vi "ReadAndParseXML.vi"() -> (0 "Mode XML Elements":string, 2 "XML Elements":string[](array[string]))   [LabVIEW 2023, in "GettingStartedWindow.lvlib"]
uses:
  <resource>/modes/FRC/GettingStartedWindow.lvlib
  <resource>/modes/FRC/LocalizedStrings.vi
panel:
  out "error out":errorcluster
  in  "error in (no error)":errorcluster
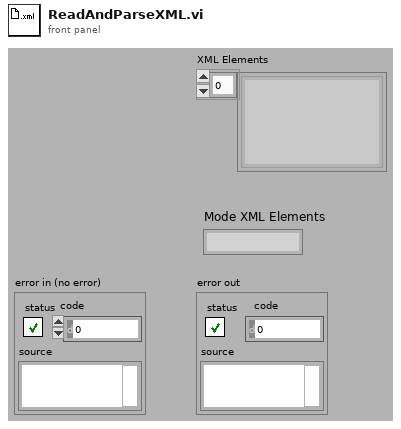
[diagram p1: front panel]
types:
  T1 = enum16{"open", "replace", "create", "open or create", "replace or create", "replace or create with confirmation"}
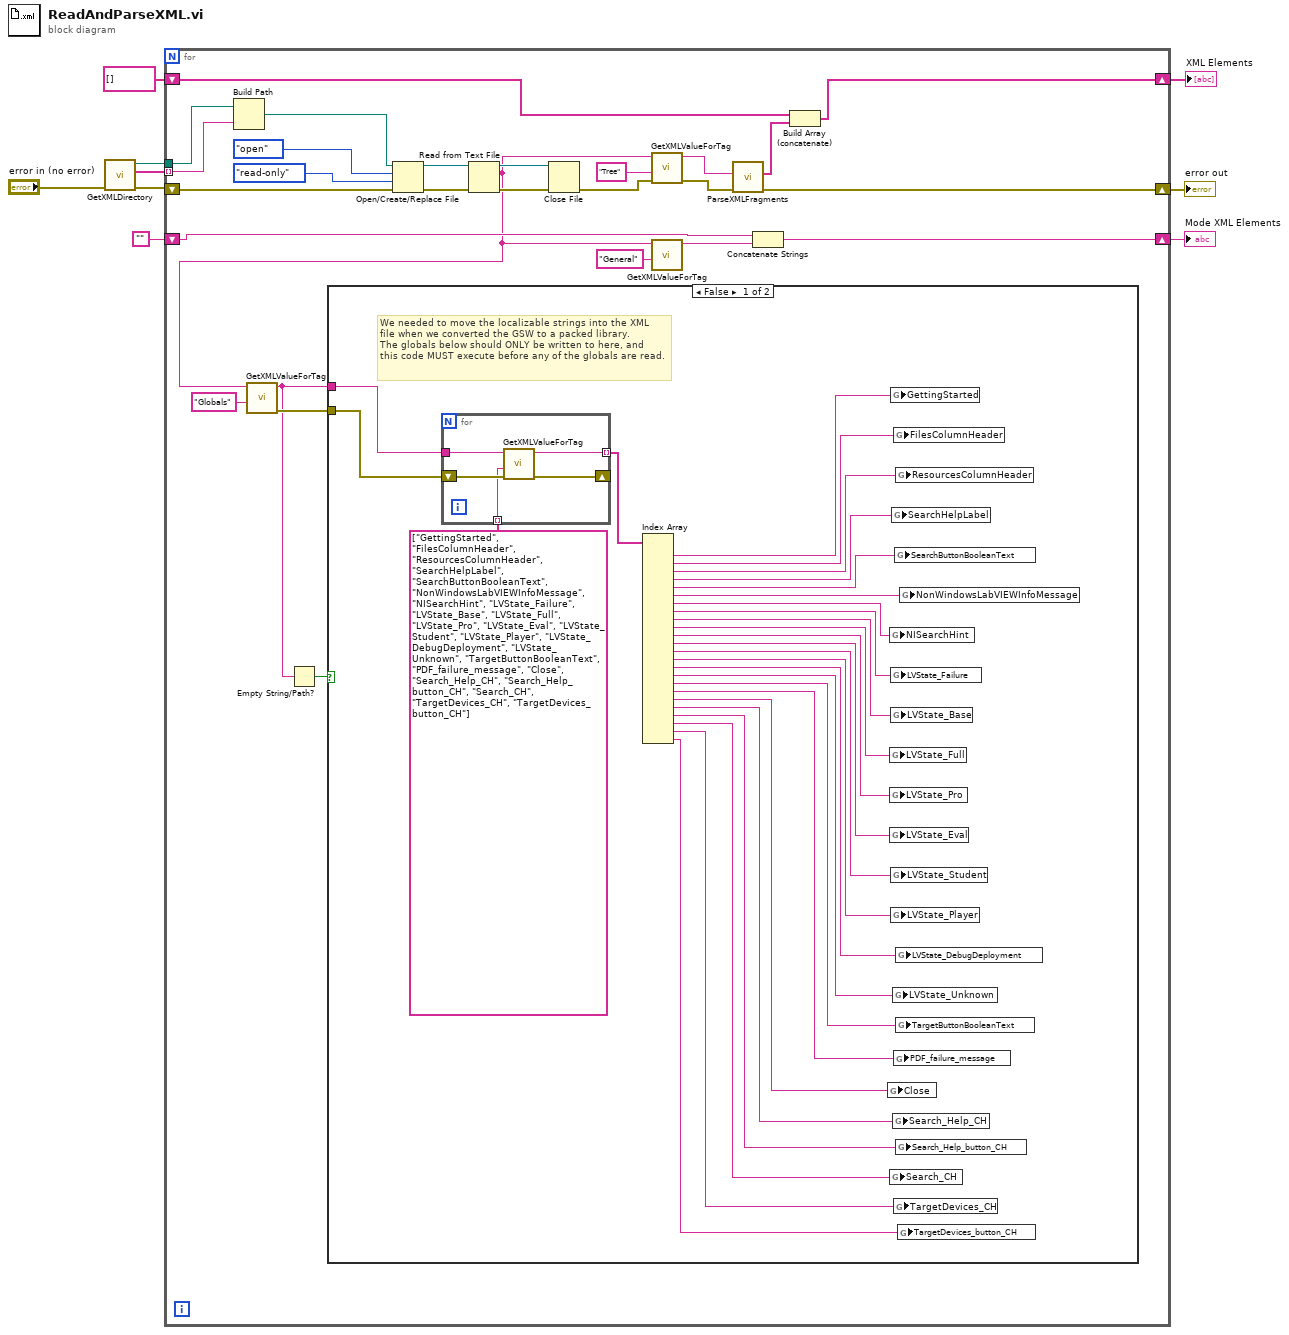
[diagram p0: block diagram]
diagram:
  n1 = call <resource>:"GetXMLDirectory.vi"("error in (no error)"="error in (no error)") -> ("error out"=w4:errorcluster, "filenames"=w5:string[], "path out"=w6:path)  [unwired: 8 out]
  n2 = for {
    shift-right: [w35] -> w9
    shift-left: w4 -> [w27]
    tunnel: w5 -> [w25] mode=indexing
    tunnel: w6 -> [w26]
    shift-right: [w19] -> w8
    shift-left: string[] [] -> [w20]
    shift-right: [w15] -> w1
    shift-left: "" -> [w17]
    n3 = Build Path(base path=w26, name or relative path=w25) -> (appended path=w24:path)
    n4 = Open/Create/Replace File(file path (use dialog)=w24, error in=w27, operation (0:open)=T1."open", access (0:read/write)=enum16{"read/write", "read-only", "write-only"}."read-only") -> (refnum out=w30:refnum<file>, error out=w31:errorcluster)  [unwired: 3 out]
    n5 = Read from Text File(file (use dialog)=w30, error in=w31) -> (refnum out=w36:refnum<file>, text=w14:string, error out=w34:errorcluster)  [unwired: 3 out]
    n6 = call <resource>:"GetXMLValueForTag.vi"("tag"="Globals", "XML"=w14) -> ("error out"=w12:errorcluster, "value"=w10:string)  [unwired: 2 in, 6 out]
    n7 = Empty String/Path?(string/path=w10) -> (empty?=w11:bool)
    n8 = case shown="False" w11 {
      tunnel: w12 -> [w64 _]
      tunnel: w10 -> [w63 _]
      frame False {
        # "We needed to move the localizable strings into the XML\nfile when we converted the GSW to a packed library.\nThe globals below should ONLY be written to here, and\nthis code MUST execute before any of the globals are read."
        n9 = for {
          tunnel: w63 -> [w68]
          shift-right: [w67] -> _
          shift-left: w64 -> [w69]
          tunnel: [w66] -> w61 mode=indexing
          tunnel: string[] ["GettingStarted", "FilesColumnHeader", "ResourcesColumnHeader", "SearchHelpLabel", "SearchButtonBooleanText", "NonWindowsLabVIEWInfoMessage", "NISearchHint", "LVState_Failure", "LVState_Base", "LVState_Full", "LVState_Pro", "LVState_Eval", "LVState_Student", "LVState_Player", "LVState_DebugDeployment", "LVState_Unknown", "TargetButtonBooleanText", "PDF_failure_message", "Close", "Search_Help_CH", "Search_Help_button_CH", "Search_CH", "TargetDevices_CH", "TargetDevices_button_CH"] -> [w65] mode=indexing
          n10 = call <resource>:"GetXMLValueForTag.vi"("error in (no error)"=w69, "tag"=w65, "XML"=w68) -> ("error out"=w67:errorcluster, "value"=w66:string)  [unwired: 1 in, 6 out]
        }
        n11 = Index Array(array=w61) -> (element #1=w60:string, element #2=w59:string, element #3=w58:string, element #4=w57:string, element #5=w56:string, element #6=w55:string, element #7=w54:string, element #8=w53:string, element #9=w52:string, element #10=w51:string, element #11=w50:string, element #12=w49:string, element #13=w48:string, element #14=w47:string, element #15=w46:string, element #16=w45:string, element #17=w44:string, element #18=w43:string, element #19=w42:string, element #20=w41:string, element #21=w40:string, element #22=w39:string, element #23=w38:string, element #24=w37:string)  [unwired: 24 in]
        n12 = global write "LocalizedStrings.vi" "Close"(w42) -> ()
        n13 = global write "LocalizedStrings.vi" "NISearchHint"(w54) -> ()
        n14 = global write "LocalizedStrings.vi" "LVState_Full"(w51) -> ()
        n15 = global write "LocalizedStrings.vi" "LVState_Pro"(w50) -> ()
        n16 = global write "LocalizedStrings.vi" "LVState_Eval"(w49) -> ()
        n17 = global write "LocalizedStrings.vi" "Search_CH"(w39) -> ()
        n18 = global write "LocalizedStrings.vi" "GettingStarted"(w60) -> ()
        n19 = global write "LocalizedStrings.vi" "LVState_Failure"(w53) -> ()
        n20 = global write "LocalizedStrings.vi" "LVState_Base"(w52) -> ()
        n21 = global write "LocalizedStrings.vi" "LVState_Student"(w48) -> ()
        n22 = global write "LocalizedStrings.vi" "LVState_Player"(w47) -> ()
        n23 = global write "LocalizedStrings.vi" "SearchHelpLabel"(w57) -> ()
        n24 = global write "LocalizedStrings.vi" "LVState_Unknown"(w45) -> ()
        n25 = global write "LocalizedStrings.vi" "Search_Help_CH"(w41) -> ()
        n26 = global write "LocalizedStrings.vi" "FilesColumnHeader"(w59) -> ()
        n27 = global write "LocalizedStrings.vi" "PDF_failure_message"(w43) -> ()
        n28 = global write "LocalizedStrings.vi" "TargetDevices_CH"(w38) -> ()
        n29 = global write "LocalizedStrings.vi" "SearchButtonBooleanText"(w56) -> ()
        n30 = global write "LocalizedStrings.vi" "ResourcesColumnHeader"(w58) -> ()
        n31 = global write "LocalizedStrings.vi" "LVState_DebugDeployment"(w46) -> ()
        n32 = global write "LocalizedStrings.vi" "TargetButtonBooleanText"(w44) -> ()
        n33 = global write "LocalizedStrings.vi" "Search_Help_button_CH"(w40) -> ()
        n34 = global write "LocalizedStrings.vi" "TargetDevices_button_CH"(w37) -> ()
        n35 = global write "LocalizedStrings.vi" "NonWindowsLabVIEWInfoMessage"(w55) -> ()
      }
      frame True {
      }
    }
    n36 = Close File(refnum=w36, error in=w34) -> (error out=w23:errorcluster)  [unwired: 1 out]
    n37 = call <resource>:"GetXMLValueForTag.vi"("error in (no error)"=w23, "tag"="Tree", "XML"=w14) -> ("error out"=w22:errorcluster, "value"=w29:string)  [unwired: 1 in, 6 out]
    n38 = call <resource>:"GetXMLValueForTag.vi"("tag"="General", "XML"=w14) -> ("value"=w16:string)  [unwired: 2 in, 7 out]
    n39 = call <vilib>:"ParseXMLFragments.vi"("error in (no error)"=w22, "XML in"=w29) -> ("error out"=w35:errorcluster, "XML Elements"=w21:string[])  [unwired: 8 out]
    n40 = Concatenate Strings(w17, w16) -> (w15:string)
    n41 = Build Array (concatenate)(w20, w21) -> (w19:string[])
  }
  "error out" <- w9
  "XML Elements" <- w8
  "Mode XML Elements" <- w1
